vi "Check Action.vi"(6 "HRS Time":dbl, 7 "Values In":dbl[](array[numeric]), 8 "error in (no error)":errorcluster, 11 "Valve in":refnum<class "DiscreteRangeControl.lvclass">) -> (0 "error out":errorcluster, 2 "Actions":T1[](array[typedef]), 3 "Valve out":refnum<class "DiscreteRangeControl.lvclass">, 5 "Values":dbl[](array[numeric]))   [LabVIEW 2020, in "VolatusControl.lvlib" / "DiscreteRangeControl.lvclass"]
uses:
  DiscreteRangeControl.lvclass
  Control Action.ctl
  Volatus/MessageQ/MessageQ.lvclass
  DiscreteRangeControl.lvclass/DiscreteRangeControl.ctl
  State.ctl
  PV Calc/PV Calc.lvclass
  VolatusControl.lvlib
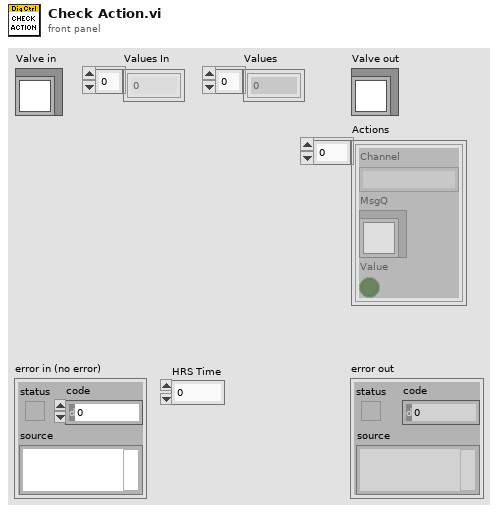
[diagram p1: front panel]
types:
  T1 = typedef "VolatusControl.lvlib/Control Action.ctl" = cluster{"Channel":string, "MsgQ":refnum<class "MessageQ.lvclass">, "Value":bool}
  T2 = typedef "VolatusControl.lvlib/DiscreteRangeControl.lvclass/State.ctl" = enum16{"Idle", "Start", "Run", "Stop"}
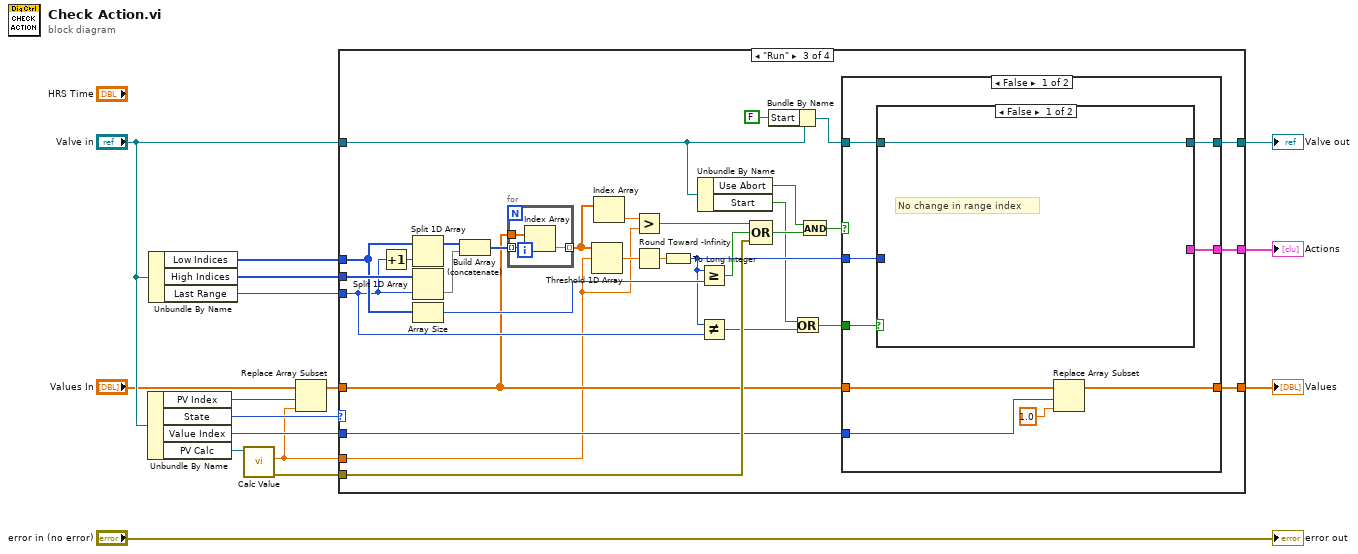
[diagram p0: block diagram]
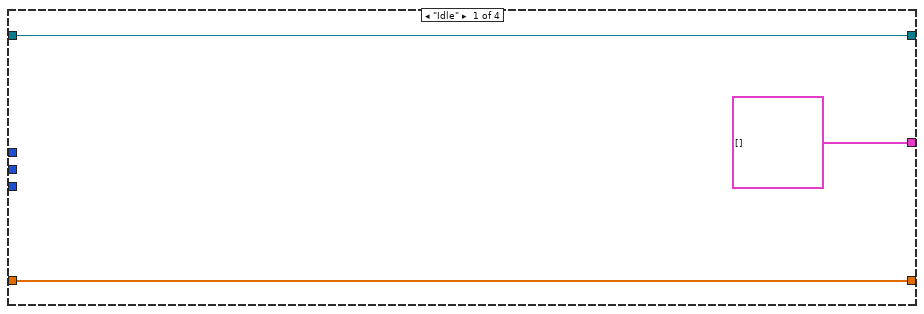
[diagram p2: hidden frame]
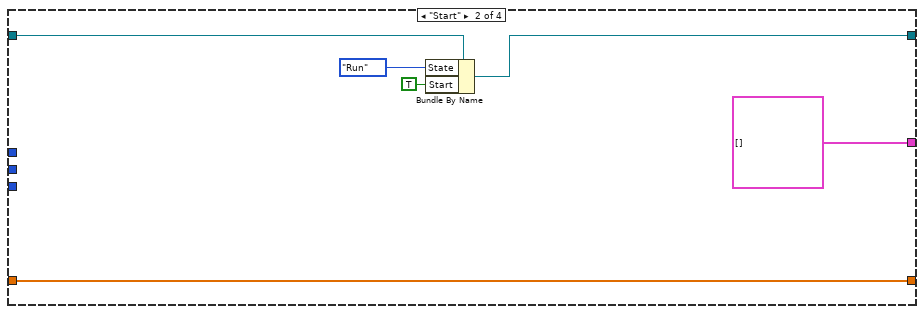
[diagram p3: hidden frame]
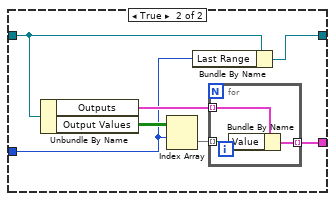
[diagram p4: hidden frame]
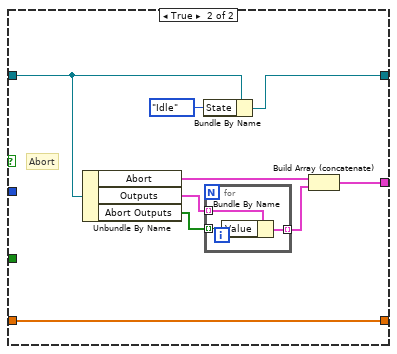
[diagram p5: hidden frame]
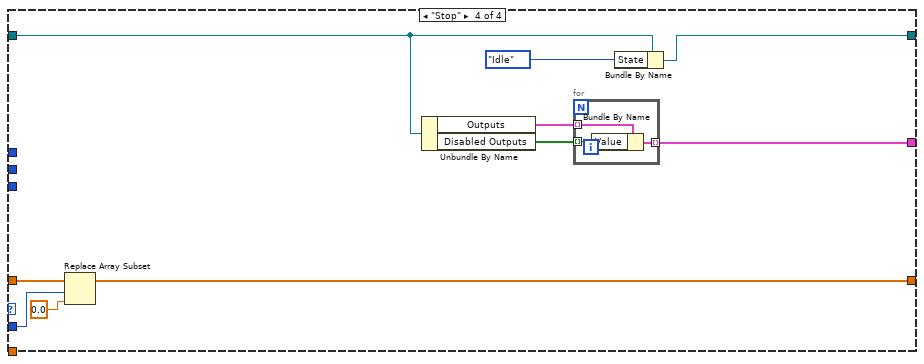
[diagram p6: hidden frame]
diagram:
  n1 = Unbundle By Name("Valve in") -> ("PV Index"=w4:i32, "State"=w7:T2, "Value Index"=w9:i32, "PV Calc"=w3:refnum<class "PV Calc.lvclass">)
  n2 = Unbundle By Name("Valve in") -> ("Low Indices"=w14:i32[], "High Indices"=w15:i32[], "Last Range"=w13:i32)
  n3 = call "Calc Value.vi"("PV Calc in"=w3) -> ("error out"=w2:errorcluster, "Value"=w1:dbl)  [unwired: 8 in, 1 out]
  n4 = Replace Array Subset(array="Values In", new element=w1, index=w4) -> (w5:dbl[])
  n5 = case shown="\"Run\"" w7 {
    tunnel: w15 -> [_ _ w55 _]
    tunnel: w5 -> [w18 w23 w27 w101]
    tunnel: w14 -> [_ _ w50 _]
    tunnel: w13 -> [_ _ w42 _]
    tunnel: [w18 w23 w40 w98] -> w12
    tunnel: [w19 w22 w39 w93] -> w11
    tunnel: "Valve in" -> [w19 w25 w35 w97]
    tunnel: w9 -> [_ _ w33 w100]
    tunnel: [T1[] [] T1[] [] w37 w94] -> w8
    tunnel: w2 -> [_ _ w56 _]
    tunnel: w1 -> [_ _ w26 _]
    frame "Idle" {
    }
    frame "Start" {
      n6 = Bundle By Name(cluster=w25, "State"=State."Run", "Start"=TRUE) -> (w22:refnum<class "DiscreteRangeControl.lvclass">)
    }
    frame "Run" {
      n7 = Increment(x=w42) -> (x+1=w51:i32)
      n8 = Split 1D Array(array=w50, index=w51) -> (first subarray=w54:i32[])  [unwired: 1 out]
      n9 = Split 1D Array(array=w55, index=w42) -> (second subarray=w53:i32[])  [unwired: 1 out]
      n10 = Array Size(array=w50) -> (size(s)=w46:i32)
      n11 = Build Array (concatenate)(w54, w53) -> (w52:i32[])
      n12 = for {
        tunnel: w27 -> [w59]
        tunnel: w52 -> [w58] mode=indexing
        tunnel: [w57] -> w49 mode=indexing
        n13 = Index Array(array=w59, index=w58) -> (element=w57:dbl)
      }
      n14 = Threshold 1D Array(2:w26, 3:w49) -> (0:w45:dbl)  [unwired: 1 in]
      n15 = Index Array(array=w49) -> (element=w48:dbl)  [unwired: 1 in]
      n16 = Greater?(x=w48, y=w26) -> (0:w47:bool)
      n17 = Round Toward -Infinity(1:w45) -> (0:w44:dbl)
      n18 = To Long Integer(number=w44) -> (32bit integer=w38:i32)
      n19 = Unbundle By Name(w35) -> ("Use Abort"=w34:bool, "Start"=w30:bool)
      n20 = Greater Or Equal?(x=w38, y=w46) -> (x >= y?=w43:bool)
      n21 = Not Equal?(x=w38, y=w42) -> (x != y?=w31:bool)
      n22 = Compound Arithmetic op=OR(w47, w43, w56) -> (w41:bool)
      n23 = Bundle By Name(cluster=w35, "Start"=FALSE) -> (w29:refnum<class "DiscreteRangeControl.lvclass">)
      n24 = Or(x=w30, y=w31) -> (x .or. y?=w32:bool)
      n25 = And(x=w34, y=w41) -> (x .and. y?=w36:bool)
      n26 = case shown="False" w36 {
        tunnel: w29 -> [w62 w87]
        tunnel: w27 -> [w65 w88]
        tunnel: [w63 w88] -> w40
        tunnel: [w67 w81] -> w39
        tunnel: w38 -> [w66 _]
        tunnel: [w68 w82] -> w37
        tunnel: w32 -> [w64 _]
        tunnel: w33 -> [w60 _]
        frame False {
          n27 = case shown="False" w64 {
            tunnel: [_ w73] -> w68
            tunnel: w62 -> [w69 w72]
            tunnel: [w69 w71] -> w67
            tunnel: w66 -> [_ w70]
            frame False {
              # "No change in range index"
            }
            frame True {
              n28 = Unbundle By Name(w72) -> ("Outputs"=w74:T1[], "Output Values"=w76:bool[][])
              n29 = Index Array(array=w76, index (row)=w70) -> (element=w75:bool[])  [unwired: 1 in]
              n30 = Bundle By Name(cluster=w72, "Last Range"=w70) -> (w71:refnum<class "DiscreteRangeControl.lvclass">)
              n31 = for {
                tunnel: w75 -> [w78] mode=indexing
                tunnel: w74 -> [w79] mode=indexing
                tunnel: [w77] -> w73 mode=indexing
                n32 = Bundle By Name(cluster=w79, "Value"=w78) -> (w77:T1)
              }
            }
          }
          n33 = Replace Array Subset(array=w65, new element=1.0 ("new element/subarray"), index=w60) -> (w63:dbl[])
        }
        frame True {
          # "Abort"
          n34 = Unbundle By Name(w87) -> ("Abort"=w84:T1, "Outputs"=w86:T1[], "Abort Outputs"=w85:bool[])
          n35 = Bundle By Name(cluster=w87, "State"=State."Idle") -> (w81:refnum<class "DiscreteRangeControl.lvclass">)
          n36 = for {
            tunnel: w86 -> [w91] mode=indexing
            tunnel: w85 -> [w90] mode=indexing
            tunnel: [w89] -> w83 mode=indexing
            n37 = Bundle By Name(cluster=w91, "Value"=w90) -> (w89:T1)
          }
          n38 = Build Array (concatenate)(w84, w83) -> (w82:T1[])
        }
      }
    }
    frame "Stop" {
      n39 = Replace Array Subset(array=w101, new element=0.0 ("new element/subarray"), index=w100) -> (w98:dbl[])
      n40 = Unbundle By Name(w97) -> ("Outputs"=w96:T1[], "Disabled Outputs"=w95:bool[])
      n41 = for {
        tunnel: w96 -> [w104] mode=indexing
        tunnel: w95 -> [w103] mode=indexing
        tunnel: [w102] -> w94 mode=indexing
        n42 = Bundle By Name(cluster=w104, "Value"=w103) -> (w102:T1)
      }
      n43 = Bundle By Name(cluster=w97, "State"=State."Idle") -> (w93:refnum<class "DiscreteRangeControl.lvclass">)
    }
  }
  "Valve out" <- w11
  "Actions" <- w8
  "Values" <- w12
  "error out" <- "error in (no error)"
